vi "Create Frame (empty).vi"(6 "stylename":string, 8 "error in (no error)":errorcluster, 11 "ooWriter in":refnum<class "ooWriter.lvclass">) -> (0 "error out":errorcluster, 2 "Frame (graphic)":refnum<k24>, 3 "ooWriter out":refnum<class "ooWriter.lvclass">)   [LabVIEW 2009, in "ooWriter.lvclass"]
uses:
  ooWriter.lvclass
  C:/Projets/LAVAG/OpenOfficeRGT/AODL/DLLs/AODL.dll
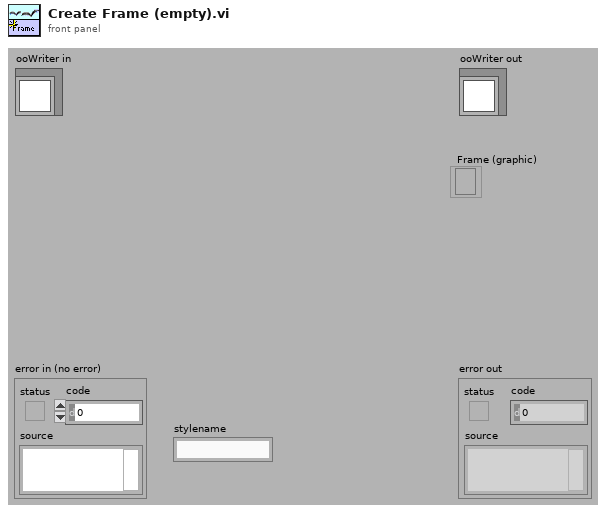
[diagram p1: front panel]
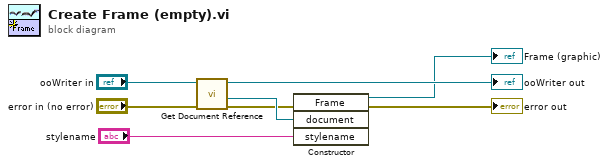
[diagram p0: block diagram]
diagram:
  n1 = call-dynamic "Get Document Reference.vi"("error in (no error)"="error in (no error)", "ooDocument in"="ooWriter in") -> ("error out"=w1:errorcluster, "Document"=w2:refnum<k24>, "ooDocument out"=→"ooWriter out":refnum<class "ooWriter.lvclass">)  [unwired: 7 in]
  n2 = constructor class="Frame"(error in=w1, "document"=w2, "stylename"="stylename") -> (reference out=→"Frame (graphic)":refnum<k24>, error out=→"error out":errorcluster)  [unwired: 2 in, 3 out]
